vi "query LTE Uplink Channel Number.vi"(8 "error in (no error)":errorcluster, 9 "UL Channel Arguments":T2, 11 "Anritsu Call Box in":refnum<class "Anritsu Call Box.lvclass">) -> (0 "error out":errorcluster, 2 "UL Channel Info":T1, 3 "Anritsu Call Box out":refnum<class "Anritsu Call Box.lvclass">)   [LabVIEW 2023, in "ANRITSU Call Box.lvlib" / "Anritsu Call Box.lvclass"]
uses:
  Anritsu Call Box.lvclass
  Type Definition/LTE Uplink Channel Number Target.ctl
  ANRITSU Call Box.lvlib
  Type Definition/LTE Uplink Channel Number Info.ctl
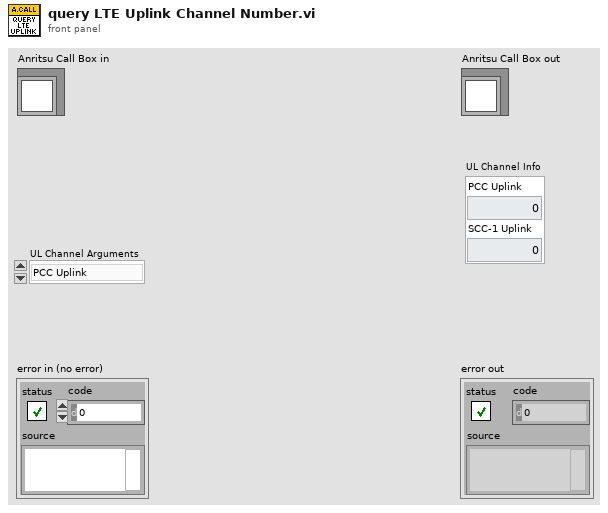
[diagram p1: front panel]
types:
  T1 = typedef "ANRITSU Call Box.lvlib/LTE Uplink Channel Number Info.ctl" = cluster{"PCC Uplink":i32, "SCC-1 Uplink":i32}
  T2 = typedef "ANRITSU Call Box.lvlib/LTE Uplink Channel Number Target.ctl" = enum16{"PCC Uplink", "SCC-1 Uplink", "All"}
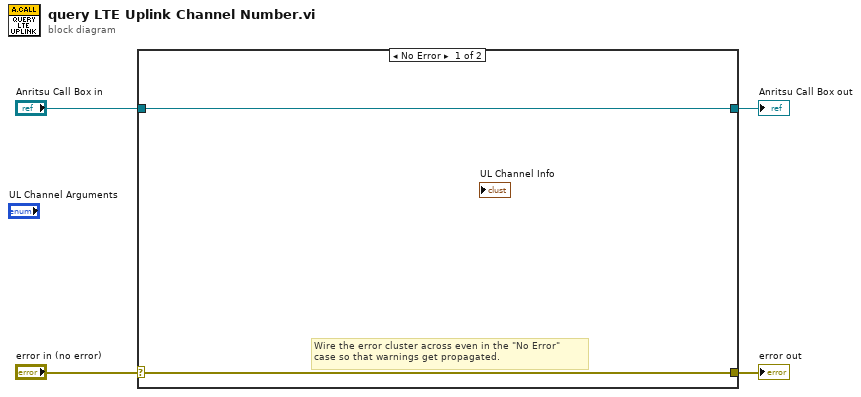
[diagram p0: block diagram]
diagram:
  n1 = case shown="No Error" "error in (no error)" {
    selector: "error in (no error)" -> [w5 w8]
    tunnel: [w5 w8] -> w3
    tunnel: [w6 w7] -> w1
    tunnel: "Anritsu Call Box in" -> [w6 w7]
    frame No Error {
      # "Wire the error cluster across even in the \"No Error\"\ncase so that warnings get propagated."
    }
    frame Error {
    }
  }
  "error out" <- w3
  "Anritsu Call Box out" <- w1
